vi "CSM - Run Script.vi"(0 "CSM Scripts":string, 1 "Current Module (\"\" to Generate an ID)":string, 5 "Sync Response Only (F)":bool, 7 "Continue If Error? (F)":bool, 9 "Wait (5000ms)":i32=5000, 11 "error in (no error)":errorcluster, 12 "Response Timeout (-2 Using Global Settings)":i32=-2) -> (4 "Response":string[](array[string]), 10 "Scripts Left":string, 15 "error out":errorcluster)   [LabVIEW 2017, in "Communicable State Machine.lvlib"]
doc: "Executes multiple CSM commands in a single batch, supporting synchronous messages, asynchronous messages, and registrations.\n\n<b>Temporary Variable Support</b>\n\nCSM - Run Script.vi supports an additional supplementary syntax to save return values to specified temporary variables for use in subsequent instructions. Use the `=>` symbol to save the return value to a variable, and variable names are case-insensitive. In subsequent instructions, you can reference the variable using the syntax `${variable name}`.\n\nExample:\n\n```\nAPI: Random -@ csm => var1\nAPI: Random -@ csm => var2\nAPI: echo >> ${var1} -@ csm\nAPI: echo >> ${var2} -@ csm\nAPI: echo >> ${var1},${var2} -@ csm\n```\n\n<b>Additional Command</b>\n\n- Wait: Wait for the specified number of milliseconds, for example `Wait: 1000` means wait 1000 milliseconds.\n\n```\nAPI: Do Something -@ csm\nWait: 1000 // Wait 1000 milliseconds, then continue to the next instruction\nAPI: Do Something Else -@ csm\n```\n\n> [!WARNING]\n> <b>Temporary Variable Support</b> and <b>Additional Command</b> are not natively supported by CSM, but are parsed and processed by CSM - Run Script.vi. Therefore, temporary variables can only be used within the same script execution and cannot be saved or passed across scripts. Wait is also not part of the CSM instructions and cannot use this syntax elsewhere.\n\n\n> [!NOTE] <b>CSM Message Target Module Description</b>\n>\n> In Normal Mode, the target module for a CSM message is the specified module name.\n> System-level modules start with a `.` in their name. The target module for a CSM message includes the `.` in the name. For example, if the requested module name is `.System`, the target module for the CSM message is `.System`.\n> In Worker Mode, the target module for a CSM message can only be the overall module name, not the node name. For example, if the requested module name is `Worker#`, the target module for the CSM message is `Worker`.\n> In Chain of Responsibility Mode, the target module for a CSM message can only be the overall module name, not the node name. For example, if the requested module name is `Chain$1`, the target module for the CSM message is `Chain`.\n> In Chain of Responsibility Mode, a message is routed directly based on handling capability and priority (smaller number = higher priority) and is not passed sequentially across nodes.\n\n\n-- <b>Controls</b> --\n- <b>Current Module (\"\" to Generate an ID)</b>: Name of the current module. If empty, a temporary ID is generated for debugging purposes to identify the location.\n- <b>CSM Scripts</b>: CSM commands to execute.\n- <b>Sync Response Only (F)</b>: Whether <b>Response</b> should include only responses from synchronous messages. Disabled by default.\n- <b>Continue If Error? (F)</b>: Whether to continue execution if an error occurs. The default is FALSE, which specifies to not continue.\n- <b>Wait (5000 ms)</b>: Timeout duration for waiting module to be alive. The default is 5000 ms.\n- <b>Response Timeout (-2 Using Global Settings)</b>: Timeout for synchronous calls. The default is -2, which uses the global setting. You can set the global timeout using the CSM - Set TMO of Sync-Reply VI.\n\n-- <b>Indicators</b> --\n- <b>Response</b>: Results returned by the script. When <b>Sync Response Only (F)</b> is enabled, this output includes only responses from synchronous messages. Otherwise, each script line, including blank lines and comments, produces one result in order. Non-synchronous commands return an empty string.\n- <b>Scripts Left</b>: Remaining unexecuted scripts."
uses:
  Communicable State Machine.lvlib
  CSM - Broadcast Message Type.ctl
  _Shared/CSM Shared.lvlib
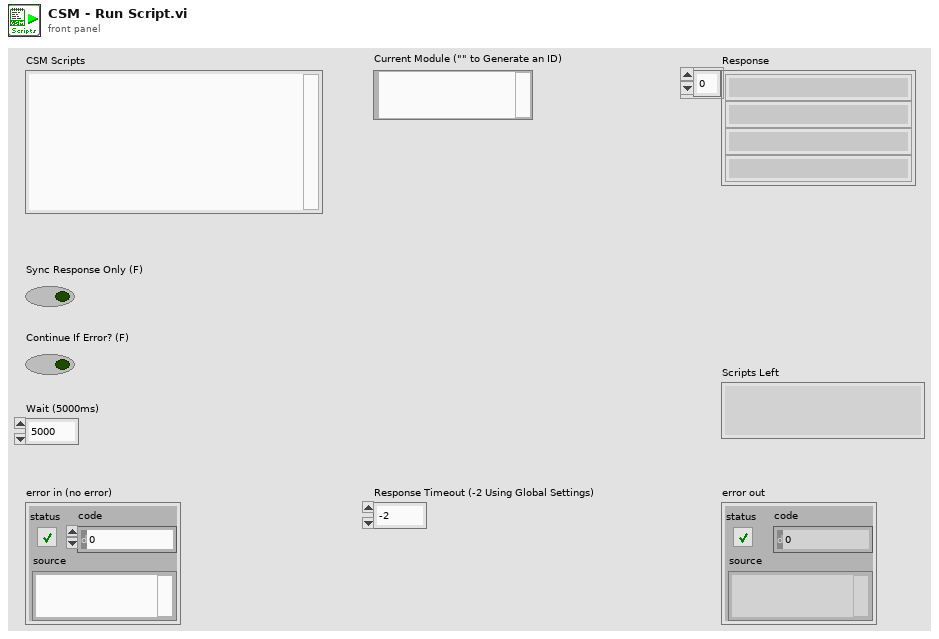
[diagram p1: front panel]
types:
  T1 = typedef "Communicable State Machine.lvlib/CSM - Broadcast Message Type.ctl" = enum16{"<Null>", "Status", "Interrupt"}
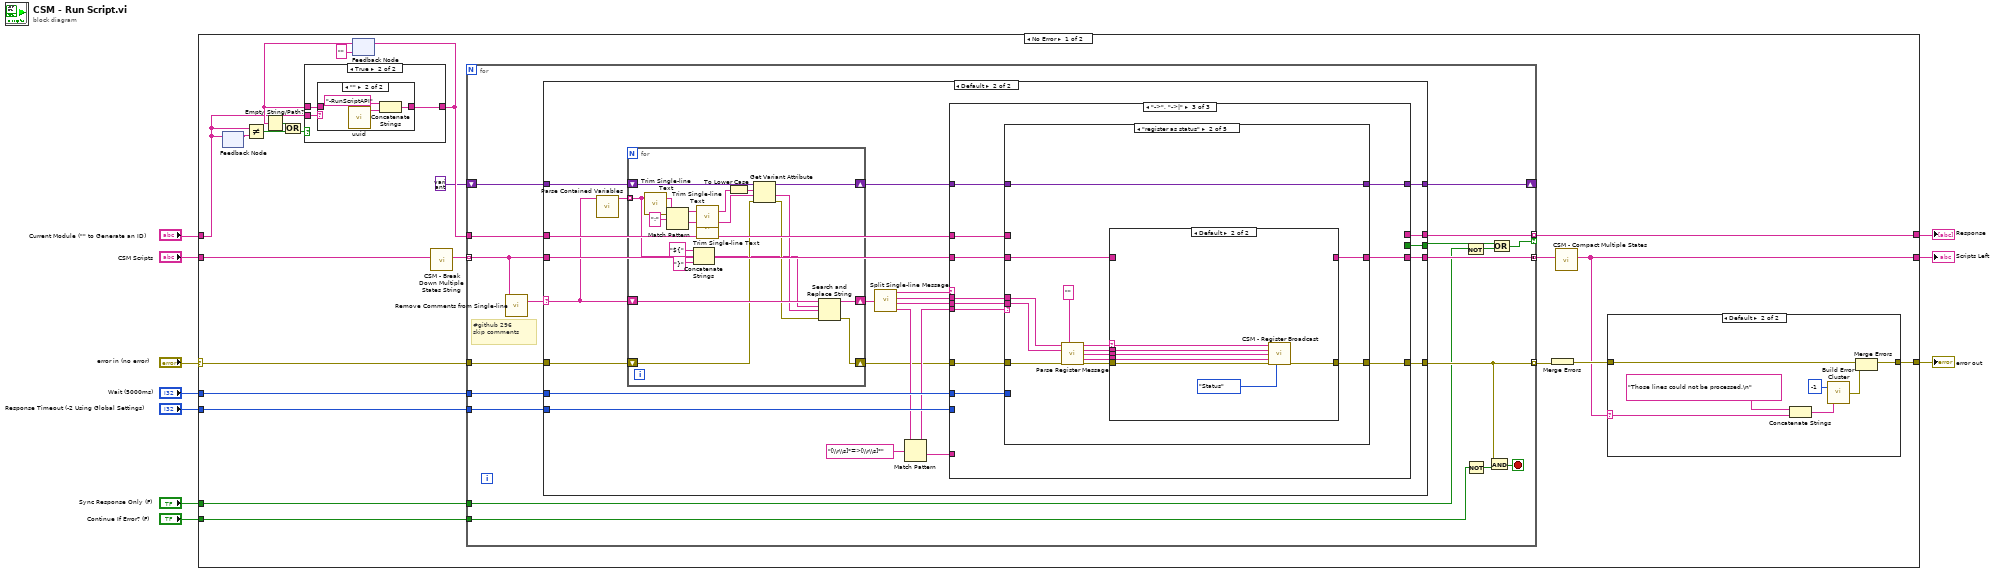
[diagram p0: block diagram]
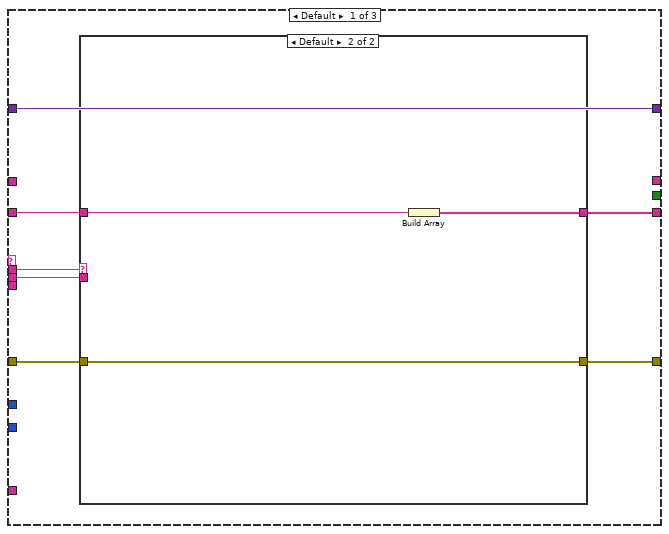
[diagram p6: hidden frame]
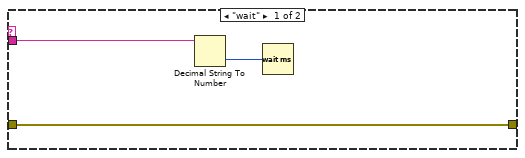
[diagram p7: hidden frame]
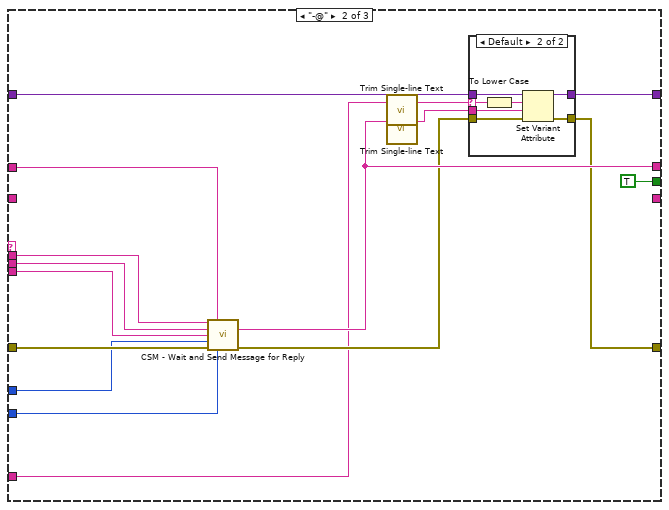
[diagram p8: hidden frame]
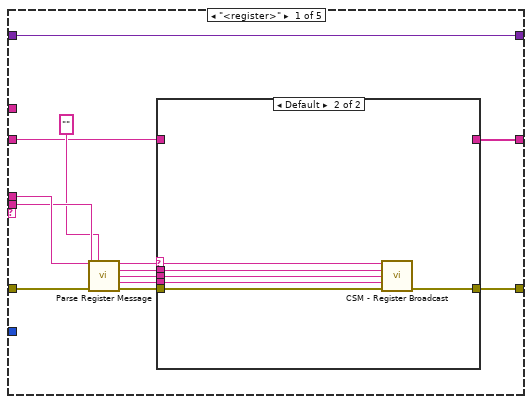
[diagram p10: hidden frame]
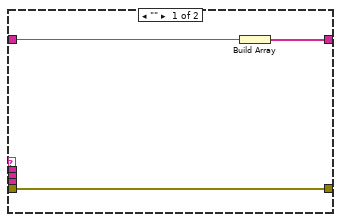
[diagram p11: hidden frame]
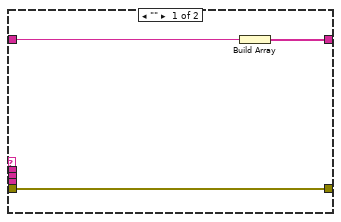
[diagram p12: hidden frame]
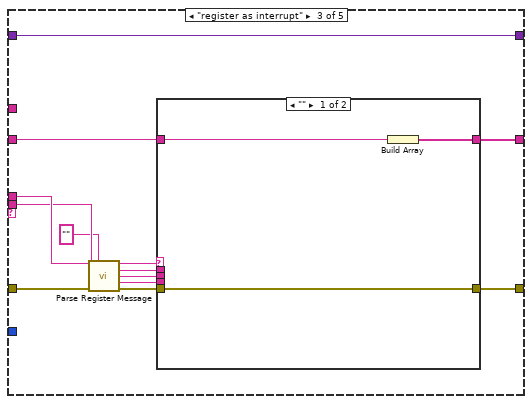
[diagram p13: hidden frame]
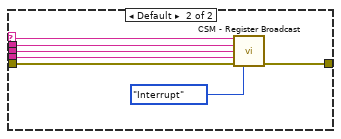
[diagram p14: hidden frame]
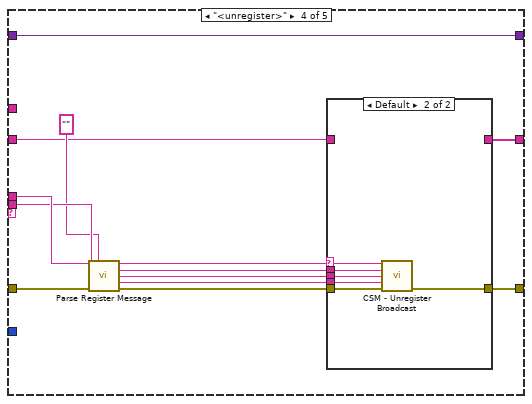
[diagram p15: hidden frame]
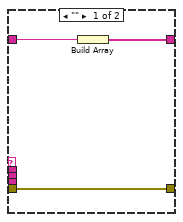
[diagram p16: hidden frame]
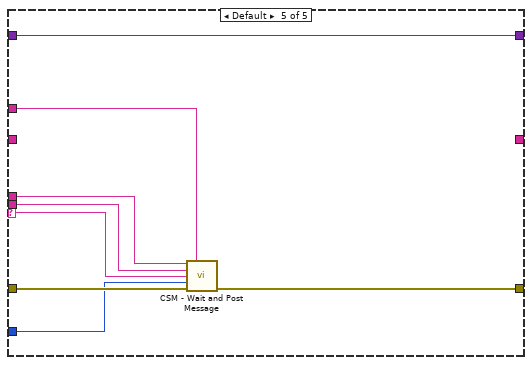
[diagram p17: hidden frame]
diagram:
  n1 = case shown="No Error" "error in (no error)" {
    selector: "error in (no error)" -> [w30 w254]
    tunnel: "CSM Scripts" -> [w29 _]
    tunnel: [w26 _] -> w8
    tunnel: [w25 w254] -> w7
    tunnel: "Current Module (\"\" to Generate an ID)" -> [w14 _]
    tunnel: "Response Timeout (-2 Using Global Settings)" -> [w24 _]
    tunnel: "Wait (5000ms)" -> [w23 _]
    tunnel: "Continue If Error? (F)" -> [w22 _]
    tunnel: [w21 _] -> w2
    tunnel: "Sync Response Only (F)" -> [w11 _]
    frame No Error {
      n2 = feedback #1() -> (w20:string)  [unwired: 1 in]
      n3 = feedback-in #1(w14) -> ()
      n4 = Not Equal?(x=w14, y=w20) -> (x != y?=w19:bool)
      n5 = feedback #2("") -> (w16:string)
      n6 = Empty String/Path?(string/path=w16) -> (empty?=w15:bool)
      n7 = Or(x=w15, y=w19) -> (x .or. y?=w17:bool)
      n8 = case shown="True" w17 {
        tunnel: w16 -> [w33 w36]
        tunnel: w14 -> [_ w35]
        tunnel: [w33 w34] -> w13
        frame False {
        }
        frame True {
          n9 = case shown="\"\"" w35 {
            selector: w35 -> [w37 _]
            tunnel: [w37 w38] -> w34
            tunnel: w36 -> [_ _]
            frame Default {
            }
            frame "" {
              n10 = call "uuid.vi"() -> ("UUID"=w39:string)  [unwired: 11 in]
              n11 = Concatenate Strings("-RunScriptAPI" ("Name (\"\" to Use UUID)"), w39) -> (w38:string)
            }
          }
        }
      }
      n12 = feedback-in #2(w13) -> ()
      n13 = call "CSM - Break Down Multiple States String.vi"("States"=w29) -> ("Multiple States"=w28:string[])  [unwired: 10 in]
      n14 = for {
        tunnel: w28 -> [w63] mode=indexing
        tunnel: w30 -> [w66]
        tunnel: [w58] -> w31 mode=indexing
        tunnel: [w64] -> w27 mode=concatenating
        tunnel: w13 -> [w62]
        tunnel: w24 -> [w61]
        tunnel: w23 -> [w60]
        tunnel: w22 -> [w57]
        tunnel: [w55] -> w21 mode=indexing if=w51
        shift-right: [w54] -> _
        shift-left: variant -> [w53]
        tunnel: w11 -> [w50]
        stop <- w59 stop-if-true
        # "#github 296\nskip comments"
        n15 = call "Remove Comments from Single-line.vi"("single-line text"=w63) -> ("single-line text without comments"=w65:string)  [unwired: 2 in]
        n16 = case shown="Default" w65 {
          selector: w65 -> [_ w72]
          tunnel: [w68 w91] -> w58
          tunnel: w66 -> [w68 w71]
          tunnel: [_ w87] -> w64
          tunnel: w63 -> [_ w86]
          tunnel: w62 -> [_ w85]
          tunnel: w61 -> [_ w84]
          tunnel: w60 -> [_ w83]
          tunnel: [_ w82] -> w55
          tunnel: [w67 w81] -> w54
          tunnel: w53 -> [w67 w76]
          tunnel: [_ w69] -> w52
          frame "" {
          }
          frame Default {
            n17 = call "Parse Contained Variables.vi"("String"=w72) -> ("Contained Variables"=w74:string[])  [unwired: 9 in, 1 out]
            n18 = for {
              shift-right: [w108] -> w75
              shift-left: w76 -> [w110]
              tunnel: w74 -> [w95] mode=indexing
              shift-right: [w101] -> w73
              shift-left: w72 -> [w100]
              shift-right: [w98] -> w70
              shift-left: w71 -> [w99]
              n19 = call "Trim Single-line Text.vi"("single-line text"=w95) -> ("trimed text"=w105:string)  [unwired: 2 in]
              n20 = Match Pattern(string=w105, regular expression=":") -> (before substring=w107:string, after substring=w106:string)  [unwired: 1 in, 2 out]
              n21 = Concatenate Strings("${" ("regular expression"), w95, "}" ("regular expression")) -> (w92:string)
              n22 = call "Trim Single-line Text.vi"("single-line text"=w107) -> ("trimed text"=w104:string)  [unwired: 2 in]
              n23 = call "Trim Single-line Text.vi"("single-line text"=w106) -> ("trimed text"=w103:string)  [unwired: 2 in]
              n24 = To Lower Case(string=w104) -> (all lower case string=w102:string)
              n25 = Get Variant Attribute(Variant=w110, name=w102, default value (empty Variant)=w103, error in=w99) -> (duplicate Variant=w108:variant, value=w96:string, error out=w97:errorcluster)  [unwired: 1 out]
              n26 = Search and Replace String(input string=w100, search string=w92, replace string=w96, error in=w97) -> (result string=w101:string, error out=w98:errorcluster)  [unwired: 4 in, 2 out]
            }
            n27 = call "Split Single-line Message.vi"("single-line text"=w73) -> ("operator"=w90:string, "state"=w88:string, "args"=w89:string, "source/target"=w79:string)  [unwired: 6 in]
            n28 = Match Pattern(string=w79, regular expression="[\\r\\s]*=>[\\r\\s]*") -> (before substring=w78:string, after substring=w77:string)  [unwired: 1 in, 2 out]
            n29 = case shown="\"->\", \"->|\"" w90 {
              tunnel: w78 -> [_ w139 w159]
              tunnel: w89 -> [w111 w138 w158]
              tunnel: w88 -> [w112 w137 w157]
              tunnel: w70 -> [w113 w136 w156]
              tunnel: [w114 w128 w155] -> w91
              tunnel: [w117 _ w154] -> w87
              tunnel: w86 -> [w116 _ w153]
              tunnel: w85 -> [_ w135 w152]
              tunnel: w84 -> [_ w134 _]
              tunnel: w83 -> [_ w133 w151]
              tunnel: [_ w130 _] -> w82
              tunnel: [w115 w131 w150] -> w81
              tunnel: w75 -> [w115 w132 w149]
              tunnel: w77 -> [_ w127 _]
              tunnel: [_ TRUE _] -> w69
              frame Default {
                n30 = case shown="Default" w112 {
                  tunnel: [_ w123] -> w117
                  tunnel: w116 -> [_ w122]
                  tunnel: [w120 w121] -> w114
                  tunnel: w113 -> [w120 w121]
                  tunnel: w111 -> [w119 _]
                  frame "wait" {
                    n31 = Decimal String To Number(string=w119) -> (number=w118:i32)  [unwired: 2 in, 1 out]
                    n32 = Wait (ms)(milliseconds to wait=w118) -> ()  [unwired: 1 out]
                  }
                  frame Default {
                    n33 = Build Array(w122) -> (w123:string[])
                  }
                }
              }
              frame "-@" {
                n34 = call "CSM - Wait and Send Message for Reply.vi"("State"=w137, "Current Module (\"\" to Generate an ID)"=w135, "Arguments (\"\")"=w138, "Target Module"=w139, "Wait (5000ms)"=w133, "Error In (No Error)"=w136, "Response Timeout (-2 Using Global Settings)"=w134) -> ("Response"=w130:string, "error out"=w129:errorcluster)  [unwired: 5 in, 2 out]
                n35 = call "Trim Single-line Text.vi"("single-line text"=w127) -> ("trimed text"=w126:string)  [unwired: 2 in]
                n36 = call "Trim Single-line Text.vi"("single-line text"=w130) -> ("trimed text"=w125:string)  [unwired: 2 in]
                n37 = case shown="Default" w126 {
                  selector: w126 -> [_ w144]
                  tunnel: w132 -> [w141 w148]
                  tunnel: [w141 w147] -> w131
                  tunnel: w129 -> [w140 w146]
                  tunnel: [w140 w145] -> w128
                  tunnel: w125 -> [_ w143]
                  frame "" {
                  }
                  frame Default {
                    n38 = To Lower Case(string=w144) -> (all lower case string=w142:string)
                    n39 = Set Variant Attribute(Variant=w148, name=w142, value=w143, error in=w146) -> (Variant out=w147:variant, error out=w145:errorcluster)  [unwired: 1 out]
                  }
                }
              }
              frame "->", "->|" {
                n40 = case shown="\"register as status\"" w159 {
                  selector: w159 -> [_ _ _ _ w253]
                  tunnel: w158 -> [w166 w187 w209 w231 w252]
                  tunnel: w157 -> [w167 w188 w210 w232 w251]
                  tunnel: w156 -> [w165 w186 w208 w230 w250]
                  tunnel: [w164 w185 w207 w229 w249] -> w155
                  tunnel: [w162 w183 w205 w227 _] -> w154
                  tunnel: w153 -> [w161 w182 w204 w226 _]
                  tunnel: w152 -> [_ _ _ _ w248]
                  tunnel: w151 -> [_ _ _ _ w247]
                  tunnel: [w160 w181 w203 w225 w246] -> w150
                  tunnel: w149 -> [w160 w181 w203 w225 w246]
                  frame "<register>" {
                    n41 = call "Parse Register Message.vi"("State"=w167, "Module Name"="", "Args"=w166) -> ("Target"=w171:string, "Source"=w170:string, "Status"=w169:string, "Api"=w168:string)  [unwired: 8 in, 1 out]
                    n42 = case shown="Default" w171 {
                      selector: w171 -> [_ w180]
                      tunnel: w170 -> [_ w179]
                      tunnel: w169 -> [_ w178]
                      tunnel: w168 -> [_ w177]
                      tunnel: w165 -> [w174 w176]
                      tunnel: [w174 w175] -> w164
                      tunnel: [w172 _] -> w162
                      tunnel: w161 -> [w173 _]
                      frame "" {
                        n43 = Build Array(w173) -> (w172:string[])
                      }
                      frame Default {
                        n44 = call "CSM - Register Broadcast.vi"("CSM Name(Empty for Broadcast Event)"=w180, "Source CSM Name (* as Default)"=w179, "Trigger"=w178, "API (If \"\", Same as Trigger)"=w177, "Error In"=w176) -> ("error out"=w175:errorcluster)  [unwired: 9 in, 1 out]
                      }
                    }
                  }
                  frame "register as status" {
                    n45 = call "Parse Register Message.vi"("State"=w188, "Module Name"="", "Args"=w187) -> ("Target"=w192:string, "Source"=w191:string, "Status"=w190:string, "Api"=w189:string)  [unwired: 8 in, 1 out]
                    n46 = case shown="Default" w192 {
                      selector: w192 -> [_ w202]
                      tunnel: w191 -> [_ w201]
                      tunnel: w190 -> [_ w200]
                      tunnel: w189 -> [_ w199]
                      tunnel: w186 -> [w195 w198]
                      tunnel: [w195 w197] -> w185
                      tunnel: [w193 _] -> w183
                      tunnel: w182 -> [w194 _]
                      frame "" {
                        n47 = Build Array(w194) -> (w193:string[])
                      }
                      frame Default {
                        n48 = call "CSM - Register Broadcast.vi"("CSM Name(Empty for Broadcast Event)"=w202, "Source CSM Name (* as Default)"=w201, "Trigger"=w200, "API (If \"\", Same as Trigger)"=w199, "Error In"=w198, "Priority (No Change)"=CSM_-_Broadcast_Message_Type."Status") -> ("error out"=w197:errorcluster)  [unwired: 8 in, 1 out]
                      }
                    }
                  }
                  frame "register as interrupt" {
                    n49 = call "Parse Register Message.vi"("State"=w210, "Module Name"="", "Args"=w209) -> ("Target"=w214:string, "Source"=w213:string, "Status"=w212:string, "Api"=w211:string)  [unwired: 8 in, 1 out]
                    n50 = case shown="\"\"" w214 {
                      selector: w214 -> [_ w224]
                      tunnel: w213 -> [_ w223]
                      tunnel: w212 -> [_ w222]
                      tunnel: w211 -> [_ w221]
                      tunnel: w208 -> [w217 w220]
                      tunnel: [w217 w219] -> w207
                      tunnel: [w215 _] -> w205
                      tunnel: w204 -> [w216 _]
                      frame "" {
                        n51 = Build Array(w216) -> (w215:string[])
                      }
                      frame Default {
                        n52 = call "CSM - Register Broadcast.vi"("CSM Name(Empty for Broadcast Event)"=w224, "Source CSM Name (* as Default)"=w223, "Trigger"=w222, "API (If \"\", Same as Trigger)"=w221, "Error In"=w220, "Priority (No Change)"=CSM_-_Broadcast_Message_Type."Interrupt") -> ("error out"=w219:errorcluster)  [unwired: 8 in, 1 out]
                      }
                    }
                  }
                  frame "<unregister>" {
                    n53 = call "Parse Register Message.vi"("State"=w232, "Module Name"="", "Args"=w231) -> ("Target"=w236:string, "Source"=w235:string, "Status"=w234:string, "Api"=w233:string)  [unwired: 8 in, 1 out]
                    n54 = case shown="Default" w236 {
                      selector: w236 -> [_ w245]
                      tunnel: w235 -> [_ w244]
                      tunnel: w234 -> [_ w243]
                      tunnel: w233 -> [_ w242]
                      tunnel: w230 -> [w239 w241]
                      tunnel: [w239 w240] -> w229
                      tunnel: [w237 _] -> w227
                      tunnel: w226 -> [w238 _]
                      frame "" {
                        n55 = Build Array(w238) -> (w237:string[])
                      }
                      frame Default {
                        n56 = call "CSM - Unregister Broadcast.vi"("CSM Name(Empty for Broadcast Event)"=w245, "Source CSM Name (* as Default)"=w244, "Trigger"=w243, "API (\"*\" as Default)"=w242, "Error In"=w241) -> ("error out"=w240:errorcluster)  [unwired: 9 in, 1 out]
                      }
                    }
                  }
                  frame Default {
                    n57 = call "CSM - Wait and Post Message.vi"("State"=w251, "Current Module (\"\" to Generate an ID)"=w248, "Arguments (\"\")"=w252, "Target Module"=w253, "Wait (5000ms)"=w247, "Error In (No Error)"=w250) -> ("error out"=w249:errorcluster)  [unwired: 8 in, 1 out]
                  }
                }
              }
            }
          }
        }
        n58 = Not(x=w50) -> (.not. x?=w49:bool)
        n59 = Not(x=w57) -> (.not. x?=w56:bool)
        n60 = And(x=w58, y=w56) -> (x .and. y?=w59:bool)
        n61 = Or(x=w52, y=w49) -> (x .or. y?=w51:bool)
      }
      n62 = Merge Errors(w31) -> (w32:errorcluster)
      n63 = call "CSM - Compact Multiple States.vi"("Multiple States"=w27) -> ("States"=w26:string)  [unwired: 9 in]
      n64 = case shown="Default" w26 {
        selector: w26 -> [_ w44]
        tunnel: w32 -> [w41 w48]
        tunnel: [w41 w43] -> w25
        frame "" {
        }
        frame Default {
          n65 = Concatenate Strings("Those lines could not be processed.\n" ("String to Prepend to source (\"\")"), w44) -> (w45:string)
          n66 = call "Build Error Cluster.vi"("String to Prepend to Source (\"\")"=w45, "Code"=-1 ("code")) -> ("error out"=w42:errorcluster)
          n67 = Merge Errors(w48, w42) -> (w43:errorcluster)
        }
      }
    }
    frame Error {
    }
  }
  "error out" <- w7
  "Scripts Left" <- w8
  "Response" <- w2
